vi "Process Python Code.vi"(8 "error in":errorcluster, 11 "G-CLI Runner in":refnum<class "Runner.lvclass">) -> (0 "error out":errorcluster, 3 "G-CLI Runner out":refnum<class "Runner.lvclass">)   [LabVIEW 2026, in "Runner.lvlib" / "Runner.lvclass"]
doc: "Run python helpers to process python code."
uses:
  Runner.lvclass
  Type Definitions/Analysis Output--cluster.ctl
  Type Definitions/Type Definition--cluster.ctl
  Type Definitions/Parameter--cluster.ctl
  Type Definitions/Function--cluster.ctl
  Runner.lvclass/Runner.ctl
  Interfaces/ILogger/ILogger Messages/Log Msg/Log Msg.lvclass/Log Msg.ctl
  <vilib>/ActorFramework/Message Enqueuer/Message Enqueuer.lvclass/Message Enqueuer.ctl
  <vilib>/ActorFramework/Message Enqueuer/Enqueue.vi
  Interfaces/ILogger/ILogger Messages/Log Msg/Log Msg.lvclass
  <vilib>/ActorFramework/Message Priority Queue/Priority Enqueue.vi
  Interfaces/IPython Caller/IPython Caller.lvclass
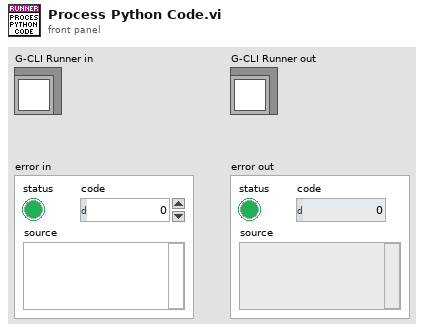
[diagram p1: front panel]
types:
  T1 = typedef "Analysis Output--cluster.ctl" = cluster{"type_definitions":T2[], "functions":T4[]}
  T2 = typedef "Type Definition--cluster.ctl" = cluster{"name":string, "fields":T3[]}
  T3 = typedef "Parameter--cluster.ctl" = cluster{"name":string, "data_type":string, "container":string, "dimensions":i32, "type_definition":string}
  T4 = typedef "Function--cluster.ctl" = cluster{"name":string, "docstring":string, "input_parameters":T3[], "output_parameters":T3[]}
  T5 = typedef "Log Entry--cluster.ctl" = cluster{"Time":timestamp, "Message":string}
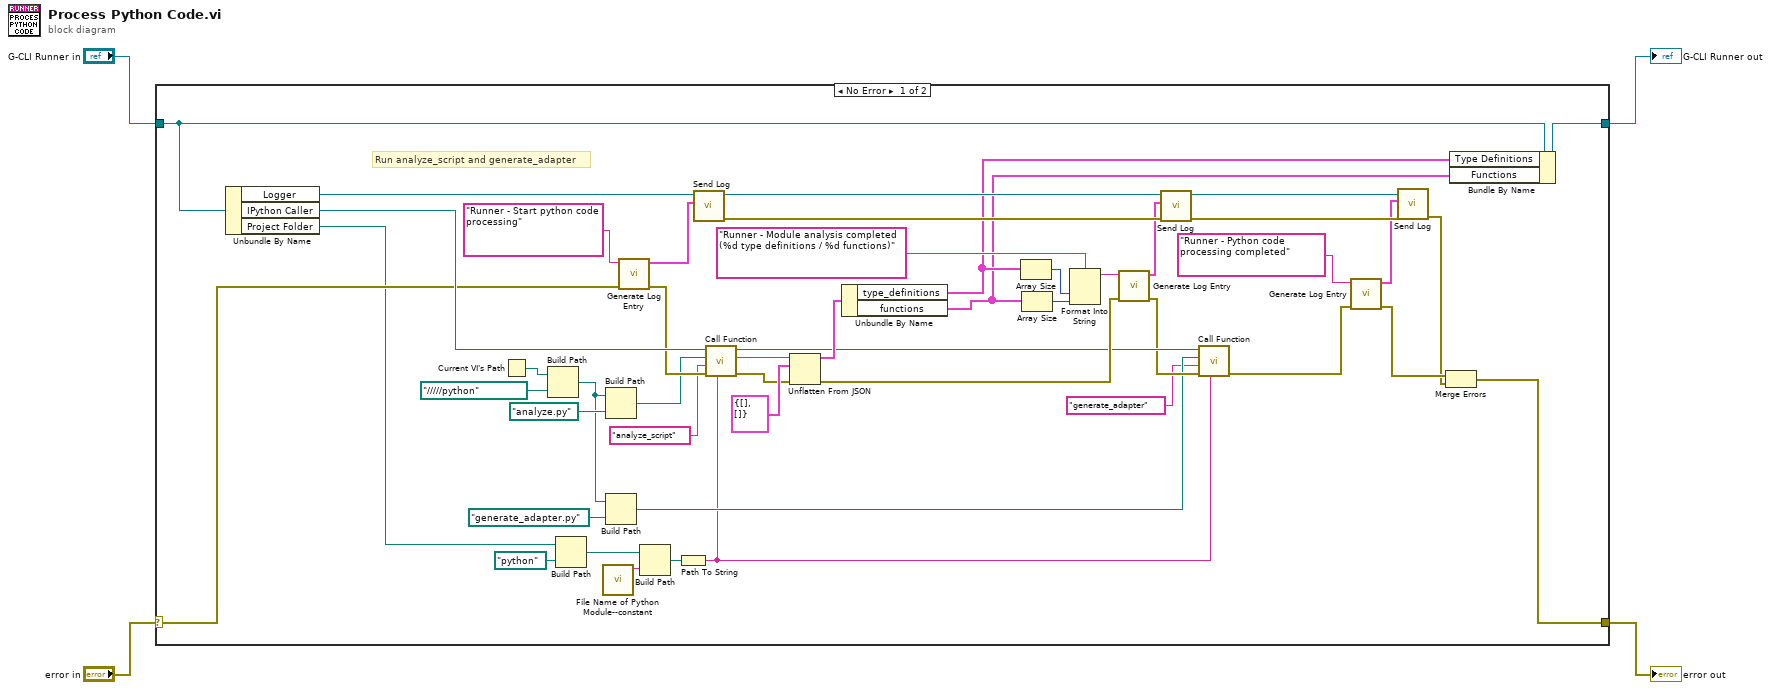
[diagram p0: block diagram]
diagram:
  n1 = case shown="No Error" "error in" {
    selector: "error in" -> [w13 w53]
    tunnel: [w51 w53] -> w4
    tunnel: "G-CLI Runner in" -> [w31 w52]
    tunnel: [w29 w52] -> w2
    frame No Error {
      # "Run analyze_script and generate_adapter"
      n2 = Unbundle By Name(w31) -> ("Logger"=w43:refnum<class "Message Enqueuer.lvclass">, "IPython Caller"=w25:refnum<class "IPython Caller.lvclass">, "Project Folder"=w8:path)
      n3 = Current VI's Path() -> (path=w12:path)
      n4 = Build Path(base path=w12, name or relative path=path "../../../../../python") -> (appended path=w9:path)
      n5 = Build Path(base path=w8, name or relative path=path "python") -> (appended path=w7:path)
      n6 = call "File Name of Python Module--constant.vi"() -> ("File Name of Python Module"=w10:string)  [unwired: 11 in]
      n7 = Build Path(base path=w9, name or relative path=path "analyze.py") -> (appended path=w23:path)
      n8 = Build Path(base path=w9, name or relative path=path "generate_adapter.py") -> (appended path=w17:path)
      n9 = call "Generate Log Entry.vi"("error in"=w13, "Message"="Runner - Start python code processing") -> ("error out"=w24:errorcluster, "Log Entry"=w42:T5)  [unwired: 8 in]
      n10 = Build Path(base path=w7, name or relative path=w10) -> (appended path=w40:path)
      n11 = Path To String(path=w40) -> (string=w15:string)
      n12 = call "Send Log.vi"("Log Entry"=w42, "Message Enqueuer"=w43) -> ("error out"=w48:errorcluster, "Message Enqueuer out"=w44:refnum<class "Message Enqueuer.lvclass">)  [unwired: 8 in]
      n13 = call-dynamic "Call Function.vi"("Input String"=w15, "error in"=w24, "Function"="analyze_script" ("function name"), "Python Script"=w23, "IPython Caller in"=w25) -> ("error out"=w20:errorcluster, "Return String"=w21:string, "IPython Caller out"=w19:refnum<class "IPython Caller.lvclass">)  [unwired: 4 in]
      n14 = Unflatten From JSON(JSON string=w21, type and defaults=T1 {"type_definitions"=[], "functions"=[]} ("Analysis Output"), error in (no error)=w20) -> (value=w38:T1, error out=w37:errorcluster)  [unwired: 4 in]
      n15 = Unbundle By Name(w38) -> ("type_definitions"=w28:T2[], "functions"=w27:T4[])
      n16 = Array Size(array=w28) -> (size(s)=w35:i32)
      n17 = Array Size(array=w27) -> (size(s)=w34:i32)
      n18 = Format Into String(format string="Runner - Module analysis completed (%d type definitions / %d functions)", w35, w34) -> (resulting string=w33:string)  [unwired: 2 in, 1 out]
      n19 = call "Generate Log Entry.vi"("error in"=w37, "Message"=w33) -> ("error out"=w18:errorcluster, "Log Entry"=w45:T5)  [unwired: 8 in]
      n20 = call "Send Log.vi"("error in (no error)"=w48, "Log Entry"=w45, "Message Enqueuer"=w44) -> ("error out"=w49:errorcluster, "Message Enqueuer out"=w47:refnum<class "Message Enqueuer.lvclass">)  [unwired: 7 in]
      n21 = call-dynamic "Call Function.vi"("Input String"=w15, "error in"=w18, "Function"="generate_adapter" ("function name"), "Python Script"=w17, "IPython Caller in"=w19) -> ("error out"=w5:errorcluster)  [unwired: 4 in, 2 out]
      n22 = call "Generate Log Entry.vi"("error in"=w5, "Message"="Runner - Python code processing completed") -> ("error out"=w50:errorcluster, "Log Entry"=w46:T5)  [unwired: 8 in]
      n23 = call "Send Log.vi"("error in (no error)"=w49, "Log Entry"=w46, "Message Enqueuer"=w47) -> ("error out"=w30:errorcluster)  [unwired: 7 in, 1 out]
      n24 = Merge Errors(w50, w30) -> (w51:errorcluster)
      n25 = Bundle By Name(cluster=w31, "Type Definitions"=w28, "Functions"=w27) -> (w29:refnum<class "Runner.lvclass">)
    }
    frame Error {
      # "Pass error without further action."
    }
  }
  "error out" <- w4
  "G-CLI Runner out" <- w2
